vi "test_NonReentrantMeasurement_MultipleMeasureCalls_ExecuteInSequence.vi"(8 "error in":errorcluster) -> (0 "error out":errorcluster, 2 "result":string, 3 "pass":bool)   [LabVIEW 2021, in "MeasurementServerTests.lvlib" / "Measurement Service Tests.lvlib"]
uses:
  Measurement Service Tests.lvlib
  Runtime/Measurements/Helpers/TypeDefs/Measurement Server User Settings.ctl
  Runtime/Measurements/Helpers/TypeDefs/Stop Server User Event.ctl
  Runtime/Measurements/Helpers/TypeDefs/Measurement Service Version.ctl
  Continuous Counting Client/controls/Measurement Configuration.ctl
  Runtime/Measurements/NI Measurement Plug-In SDK.lvlib
  Continuous Counting Client/Continuous Counting Client.lvlib
  MeasurementServerTests.lvlib
  Continuous Counting Measurement/Continuous Counting Measurement.lvclass
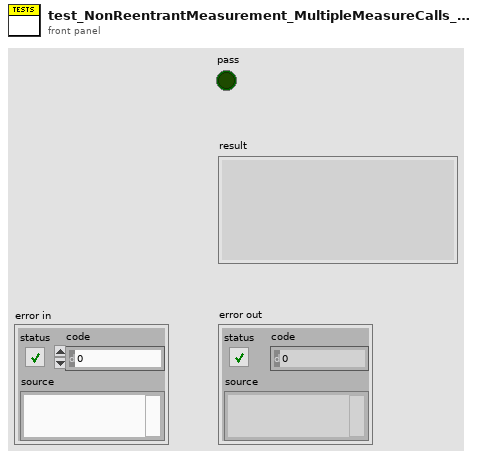
[diagram p1: front panel]
types:
  T1 = typedef "NI Measurement Plug-In SDK.lvlib/Measurement Service Version.ctl" = enum16{"V1", "V2"}
  T2 = typedef "NI Measurement Plug-In SDK.lvlib/Measurement Server User Settings.ctl" = cluster{"stop server":T3, "measurement service versions":T1[]}
  T3 = typedef "NI Measurement Plug-In SDK.lvlib/Stop Server User Event.ctl" = refnum<user-event>
  T4 = typedef "grpc-lvsupport-release.lvlib/grpcId.ctl" = u64
  T5 = typedef "MeasurementServerTests.lvlib/Measurement Service Tests.lvlib/Continuous Counting Client.lvlib/Measurement Configuration.ctl" = cluster{"ms update interval":u32}
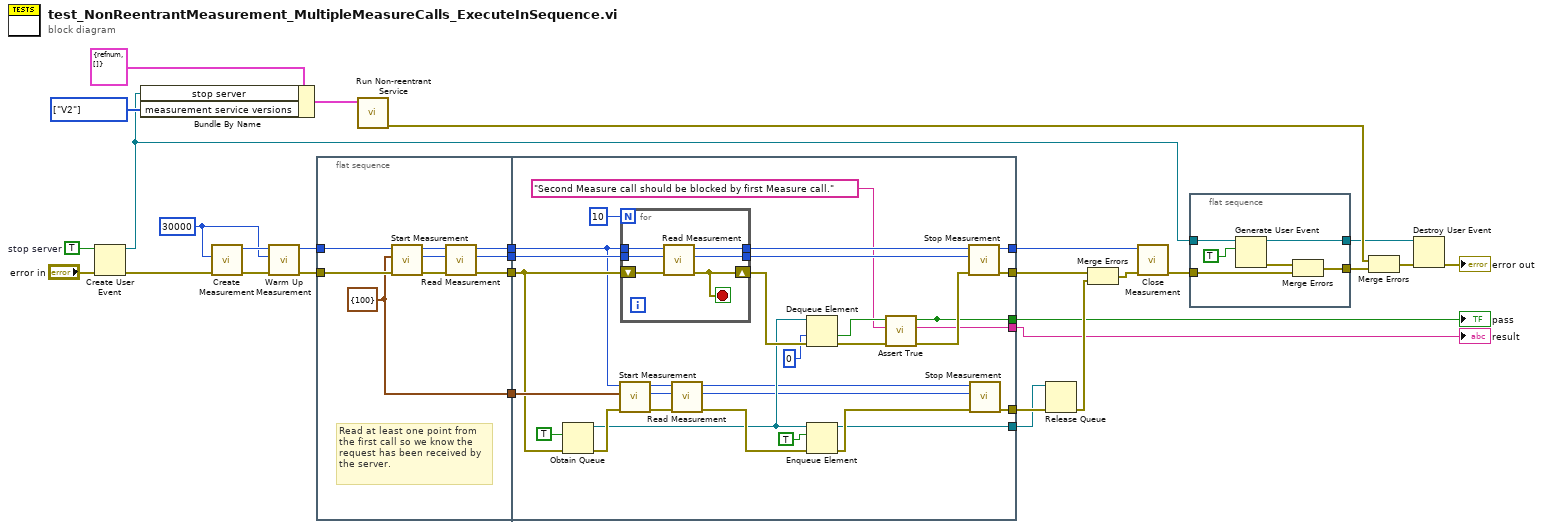
[diagram p0: block diagram]
diagram:
  w5 = 30000 ("ms timeout")
  w28 = TRUE  # stop server
  w29 = T1[] [enum."V2"] items=["V1", "V2"] ("measurement service versions")
  n1 = Create User Event(user event datatype=w28, error in="error in") -> (user event=w23:refnum<user-event>, error out=w24:errorcluster)
  n2 = Bundle By Name(cluster=T2 {"stop server"=refnum, "measurement service versions"=[]} ("server settings"), "stop server"=w23, "measurement service versions"=w29) -> (w27:T2)
  n3 = call "Create Measurement.vi"("error in"=w24, "ms timeout"=w5) -> ("error out"=w9:errorcluster, "gRPCid out"=w6:T4)  [unwired: 8 in]
  n4 = call "Warm Up Measurement.vi"("error in"=w9, "timeout (ms)"=w5, "gRPC ID"=w6) -> ("error out"=w8:errorcluster, "gRPC ID out"=w7:T4)  [unwired: 6 in, 1 out]
  n5 = flat-sequence {
    tunnel: w8 -> [w39]
    tunnel: w7 -> [w38]
    tunnel: [w35] -> w20
    tunnel: [w34] -> w19
    tunnel: [w31] -> w18
    tunnel: [w32] -> w17
    tunnel: [w63] -> w14
    tunnel: w20 -> [w60]
    tunnel: w19 -> [w40]
    tunnel: w18 -> [w69]
    tunnel: w17 -> [w64]
    tunnel: [w49] -> w16
    tunnel: [w44] -> w15
    tunnel: [w43] -> w12
    tunnel: [w41] -> _
    tunnel: [w42] -> w11
    tunnel: [w41] -> w10
    frame #0 {
      w32 = T5 {"ms update interval"=100} ("measurement configuration")
      # "Read at least one point from\nthe first call so we know the\nrequest has been received by\nthe server."
      n6 = call "Start Measurement.vi"("error in"=w39, "measurement configuration"=w32, "gRPCid in"=w38) -> ("error out"=w36:errorcluster, "call id"=w33:T4, "gRPCid out"=w37:T4)  [unwired: 6 in]
      n7 = call "Read Measurement.vi"("error in"=w36, "call id in"=w33, "gRPCid in"=w37) -> ("error out"=w35:errorcluster, "call id out"=w31:T4, "gRPCid out"=w34:T4)  [unwired: 4 in, 2 out]
    }
    frame #1 {
      n8 = Obtain Queue(element data type=TRUE, error in (no error)=w60) -> (queue out=w54:refnum<queue>, error out=w58:errorcluster)  [unwired: 3 in, 1 out]
      n9 = call "Start Measurement.vi"("error in"=w58, "measurement configuration"=w64, "gRPCid in"=w40) -> ("error out"=w67:errorcluster, "call id"=w65:T4, "gRPCid out"=w66:T4)  [unwired: 6 in]
      n10 = for {
        N: 10 -> [_]
        shift-right: [w71] -> w55
        shift-left: w60 -> [w75]
        tunnel: w40 -> [w74]
        tunnel: w69 -> [w73]
        tunnel: [w72] -> w62
        tunnel: [w70] -> w61
        stop <- w71 stop-if-true
        n11 = call "Read Measurement.vi"("error in"=w75, "call id in"=w73, "gRPCid in"=w74) -> ("error out"=w71:errorcluster, "call id out"=w70:T4, "gRPCid out"=w72:T4)  [unwired: 4 in, 2 out]
      }
      n12 = call "Read Measurement.vi"("error in"=w67, "call id in"=w65, "gRPCid in"=w66) -> ("error out"=w57:errorcluster, "call id out"=w51:T4, "gRPCid out"=w52:T4)  [unwired: 4 in, 2 out]
      n13 = Dequeue Element(queue=w54, timeout in ms (-1)=0, error in (no error)=w55) -> (timed out?=w46:bool, error out=w48:errorcluster)  [unwired: 2 out]
      n14 = Enqueue Element(queue=w54, element=TRUE, error in (no error)=w57) -> (queue out=w44:refnum<queue>, error out=w50:errorcluster)  [unwired: 1 in, 1 out]
      n15 = call "Assert True.vi"("error in"=w48, "failure message"="Second Measure call should be blocked by first Measure call.", "condition"=w46) -> ("error out"=w47:errorcluster, "message"=w42:string, "pass"=w41:bool)  [unwired: 6 in]
      n16 = call "Stop Measurement.vi"("error in"=w47, "call id"=w61, "gRPCid in"=w62) -> ("error out"=w63:errorcluster, "gRPCid out"=w43:T4)  [unwired: 7 in]
      n17 = call "Stop Measurement.vi"("error in"=w50, "call id"=w51, "gRPCid in"=w52) -> ("error out"=w49:errorcluster)  [unwired: 7 in, 1 out]
    }
  }
  n18 = call "Run Non-reentrant Service.vi"("server settings"=w27) -> ("error out"=w22:errorcluster)  [unwired: 10 in]
  n19 = Release Queue(queue=w15, error in (no error)=w16) -> (error out=w13:errorcluster)  [unwired: 1 in, 2 out]
  n20 = Merge Errors(w14, w13) -> (w25:errorcluster)
  n21 = call "Close Measurement.vi"("error in"=w25, "gRPCid in"=w12) -> ("error out"=w21:errorcluster)  [unwired: 9 in]
  n22 = flat-sequence {
    tunnel: w23 -> [w80]
    tunnel: [w79] -> w2
    tunnel: [w78] -> w4
    tunnel: w21 -> [w77]
    frame #0 {
      n23 = Generate User Event(user event=w80, event data cluster=TRUE ("event data")) -> (user event out=w79:refnum<user-event>, error out=w81:errorcluster)  [unwired: 2 in]
      n24 = Merge Errors(w81, w77) -> (w78:errorcluster)
    }
  }
  n25 = Merge Errors(w22, w4) -> (w3:errorcluster)
  n26 = Destroy User Event(user event=w2, error in=w3) -> (error out=→"error out":errorcluster)
  "pass" <- w10
  "result" <- w11
